vi "VI Script - Copy Templete MHL.vi"() -> ()   [LabVIEW 2020]
uses:
  MHL Templete/Main.vi
  MHL Templete/MHL Templete.lvlib
  support/Message Queue/Message Cluster.ctl
  support/Message Queue/Message Queue.lvlib
  support/Message Queue/All Message Queues.ctl
panel:
  in  "Message Queues":T1
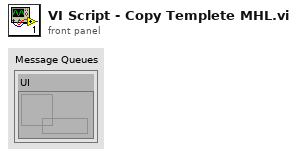
[diagram p1: front panel]
types:
  T1 = typedef "Message Queue.lvlib/All Message Queues.ctl" = cluster{"UI":refnum<queue>}
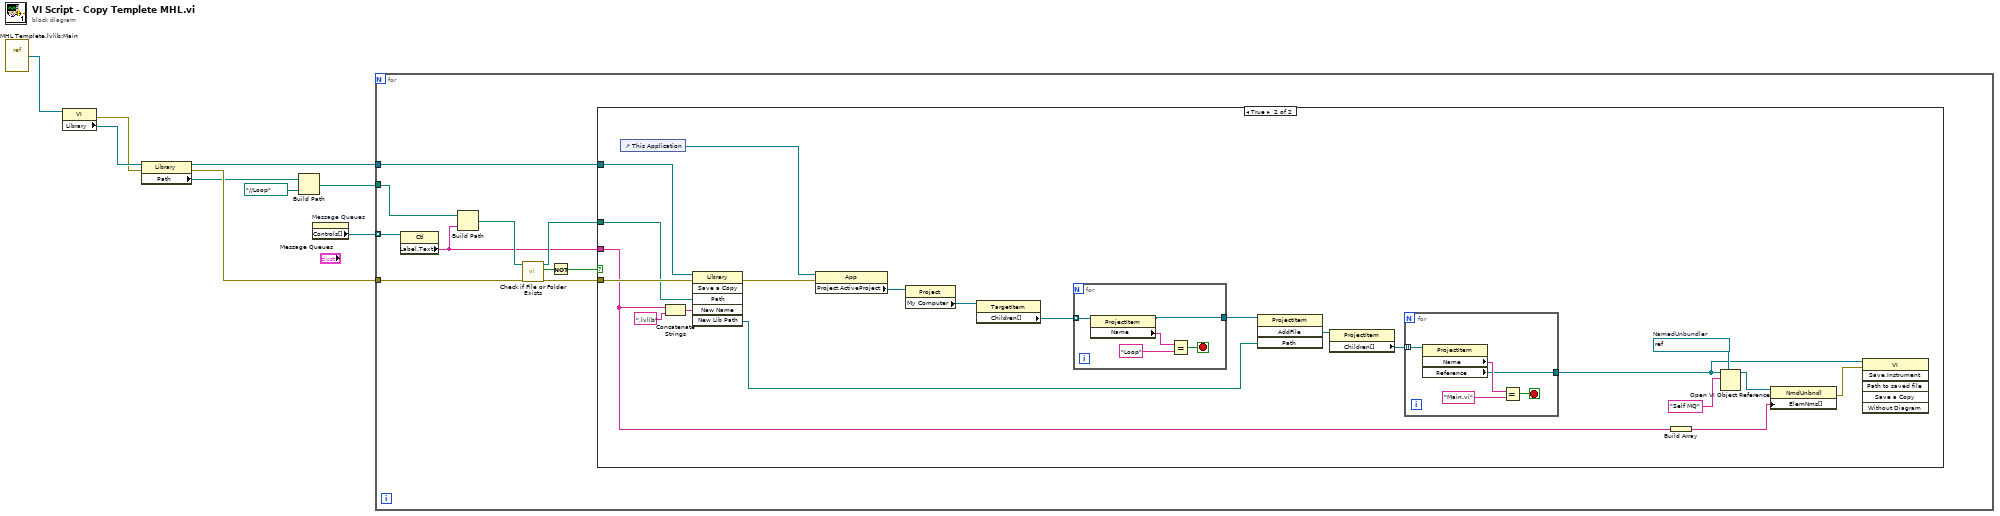
[diagram p0: block diagram]
diagram:
  n1 = vi-ref "MHL Templete.lvlib:Main.vi"() -> (w9:refnum<vi>)
  n2 = property class="VI"(reference=w9) -> (error out=w5:errorcluster, "Library"=w8:refnum<vi>)  [unwired: 1 in, 1 out]
  n3 = property class="Library"(reference=w8, error in=w5) -> (reference out=w2:refnum<vi>, error out=w4:errorcluster, "Path"=w3:path)
  n4 = Build Path(base path=w3, name or relative path=path "../../Loop") -> (appended path=w6:path)
  n5 = property on="Message Queues" class="Clust (strict)"() -> ("Controls[]"=w1:refnum<vi>[])  [unwired: 2 in, 2 out]
  n6 = for {
    tunnel: w6 -> [w19]
    tunnel: w4 -> [w17]
    tunnel: w2 -> [w11]
    tunnel: w1 -> [w10] mode=indexing
    n7 = property on="Property Node" class="Ctl"(reference=w10) -> ("Label.Text"=w12:string)  [unwired: 1 in, 2 out]
    n8 = Build Path(base path=w19, name or relative path=w12) -> (appended path=w18:path)
    n9 = call <vilib>:"Check if File or Folder Exists.vi"("error in (no error)"=w17, "path"=w18) -> ("error out"=w15:errorcluster, "file or folder exists?"=w16:bool, "dup path"=w13:path)  [unwired: 7 in]
    n10 = Not(x=w16) -> (.not. x?=w14:bool)
    n11 = case shown="True" w14 {
      tunnel: w15 -> [_ w39]
      tunnel: w13 -> [_ w37]
      tunnel: w12 -> [_ w23]
      tunnel: w11 -> [_ w38]
      frame False {
      }
      frame True {
        w25 = refnum<vi> refnum  # NamedUnbundler
        n12 = control-ref of="This Application"() -> (w36:refnum<vi>)
        n13 = Concatenate Strings(w23, ".lvlib" ("string")) -> (w33:string)
        n14 = invoke class="Library" method="Save a Copy"(reference=w38, error in=w39, "Path"=w37, "New Name"=w33) -> (error out=w35:errorcluster, "New Lib Path"=w29:path)  [unwired: 2 in, 4 out]
        n15 = property class="App"(reference=w36, error in=w35) -> ("Project.ActiveProject"=w34:refnum<vi>)  [unwired: 2 out]
        n16 = property class="Project"(reference=w34) -> ("My Computer"=w32:refnum<vi>)  [unwired: 1 in, 2 out]
        n17 = property class="TargetItem"(reference=w32) -> ("Children[]"=w31:refnum<vi>[])  [unwired: 1 in, 2 out]
        n18 = for {
          tunnel: w31 -> [w50] mode=indexing
          tunnel: [w49] -> w30
          stop <- w46 stop-if-true
          n19 = property class="ProjectItem"(reference=w50) -> (reference out=w49:refnum<vi>, "Name"=w48:string)  [unwired: 1 in, 1 out]
          n20 = Equal?(x=w48, y="Loop") -> (x = y?=w46:bool)
        }
        n21 = invoke class="ProjectItem" method="AddFile"(reference=w30, "Path"=w29) -> ("AddFile"=w28:refnum<vi>)  [unwired: 2 in, 3 out]
        n22 = property class="ProjectItem"(reference=w28) -> ("Children[]"=w27:refnum<vi>[])  [unwired: 1 in, 2 out]
        n23 = for {
          tunnel: w27 -> [w45] mode=indexing
          tunnel: [w41] -> w21
          stop <- w42 stop-if-true
          n24 = property class="ProjectItem"(reference=w45) -> ("Name"=w44:string, "Reference"=w41:refnum<vi>)  [unwired: 1 in, 2 out]
          n25 = Equal?(x=w44, y="Main.vi") -> (x = y?=w42:bool)
        }
        n26 = Build Array(w23) -> (w22:string[])
        n27 = Open VI Object Reference(7:w25, 10:"Self MQ" ("name/order"), 11:w21) -> (3:w24:refnum<vi>)  [unwired: 1 in, 1 out]
        n28 = property class="NmdUnbndl"(reference=w24, "ElemNms[]"=w22) -> (error out=w20:errorcluster)  [unwired: 1 in, 1 out]
        n29 = invoke class="VI" method="Save.Instrument"(reference=w21, error in=w20) -> ()  [unwired: 4 in, 6 out]
      }
    }
  }
